vi "Start Acquisition and Logging.vi"(8 "error in (no error)":errorcluster, 11 "Acquisition and Logging Configuration":T2={"Data Rate"=1, "Samples per Read"=0, "Number of Reads to Save"=0, "Data File Name"="", "TDMS Properties"=[], "Number of Channels"=4, "Channel Scale Array"=[0.0, 0.0, 0.0, 0.0, 1.0, 1.0, 1.0, 1.0, 1.0, 1.0, 1.0, 1.0, 1.0, 1.0, 1.0, 1.0], "Channel Names"=[], "Trigger - RMS Value"=0.0, "Trigger - Channel"=0, "Trigger - Time (Minute)"=0, "Frequency "=0, "Amplitude (0~10)"=0.0} {"Amplitude (0~10)" min=-10.0 max=10.0; "Data Rate" items=["50.000 kS/s (NI 9239)"=1, "25.000 kS/s (NI 9239)"=2, "16.667 kS/s (NI 9239)"=3, "12.500 kS/s (NI 9239)"=4, "10.000 kS/s (NI 9239)"=5, "8.333 kS/s (NI 9239)"=6, "7.143 kS/s (NI 9239)"=7, "6.250 kS/s (NI 9239)"=8, "5.556 kS/s (NI 9239)"=9, "5.000 kS/s (NI 9239)"=10, "4.545 kS/s (NI 9239)"=11, "4.167 kS/s (NI 9239)"=12, "3.846 kS/s (NI 9239)"=13, "3.571 kS/s (NI 9239)"=14, "3.333 kS/s (NI 9239)"=15, "3.125 kS/s (NI 9239)"=16, "2.941 kS/s (NI 9239)"=17, "2.778 kS/s (NI 9239)"=18, "2.632 kS/s (NI 9239)"=19, "2.500 kS/s (NI 9239)"=20, "2.381 kS/s (NI 9239)"=21, "2.273 kS/s (NI 9239)"=22, "2.174 kS/s (NI 9239)"=23, "2.083 kS/s (NI 9239)"=24, "2.000 kS/s (NI 9239)"=25, "1.923 kS/s (NI 9239)"=26, "1.852 kS/s (NI 9239)"=27, "1.786 kS/s (NI 9239)"=28, "1.724 kS/s (NI 9239)"=29, "1.667 kS/s (NI 9239)"=30, "1.613 kS/s (NI 9239)"=31]}) -> (0 "error out":errorcluster, 1 "Wait on IRQ Timeout?":bool, 2 "Total Buffer Size":i32, 3 "FPGA VI Reference Out":T5)   [LabVIEW 2016]
uses:
  controls/FPGA VI Reference.ctl
  controls/Acquisition and Logging Configuration.ctl
  <vilib>/LabVIEW Targets/FPGA/cRIO/shared/nicrio_ModuleControls/nicrio_cRIO-9239_DataRatesRing.ctl
  controls/TDMS Properties.ctl
  <vilib>/userdefined/High Color/nirio_resource_hc.ctl
  <vilib>/FPGAPlugInAG/cRIO-9068/niLvFpga_Open_cRIO-9068.vi
  <vilib>/rvi/interface/common/dynamic/niFpgaDynamicAddResources.vi
  <vilib>/FPGAPlugInAG/Dynamic/niLvFpga_Reset_Dynamic.vi
  <vilib>/Utility/error.llb/Error Cluster From Error Code.vi
  <vilib>/rvi/errors/niLvFpgaAdjustHostInterfaceError.vi
  <vilib>/rvi/interface/common/niFpgaWaitOnOcc.vi
  <vilib>/FPGAPlugInAG/Dynamic/niLvFpga_Run_Dynamic.vi
  <vilib>/RVI Host/nirviSupport.llb/nirviErrorClusterFromErrorCode.vi
  <vilib>/FPGAPlugInAG/Dynamic/niLvFpga_Close_Dynamic.vi
  <vilib>/rvi/interface/nirviOpenFPGA/nirviOpenFPGA.xnode
  FPGA Bitfiles/v1.1.10032017CSU_FPGATarget2_FPGAMain_uXAbGLR-yyg.lvbitx
  FPGA Main.vi
  <vilib>/rvi/interface/nirviMethod/nirviMethod.xnode
  <vilib>/rvi/interface/nirviReadWriteControl/nirviReadWriteControl.xnode
  <vilib>/rvi/interface/nirviCloseFPGA/nirviCloseFPGA.xnode
  <vilib>/rvi/errors/niLvFpgaMergeErrorWithErrorCode.vi
  <vilib>/rvi/interface/nirviMethod/StockFPGA_InlinedMethodWaitForSingleIRQ.vi
  <vilib>/FPGAPlugInAG/Dynamic/niLvFpga_WaitOnIrq_Dynamic.vi
  <vilib>/FPGAPlugInAG/Dynamic/niLvFpga_AcknowledgeIrq_Dynamic.vi
  <vilib>/FPGAPlugInAG/Dynamic/niLvFpga_ConfigureFifo_Dynamic.vi
  <vilib>/FPGAPlugInAG/Dynamic/niLvFpga_StartFifo_Dynamic.vi
  NiFpgaLv.dll
  <vilib>/rvi/interface/Simulation/niFpgaSimulationCallBeginRW.vi
  <vilib>/FPGAPlugInAG/Dynamic/niLvFpga_WriteFifo_Dynamic.vi
  <vilib>/FPGAPlugInAG/Dynamic/niLvFpga_ReadFifo_Dynamic.vi
panel:
  in  "Sample Frequency (Hz)":dbl=1000.0
  in  "resource name":T1="RIO0" caption="RIO Device"
  in  "stop":bool
  out "AO FIFO Empty":bool
  out "AI FIFO Full":bool
  out "AI Data":dbl[][](graph)
  # "Caso o sistema esteja Ok essa VI é chamada.\nEla contém tanto a chamada para aquisição quanto para a supervisão\nOs dados anaçógicos podem ser vistos no display em colorido.\nA VI rodada separamente funciona, mas não quando for chamada dentro do programa principal \"RT Main.vi\""
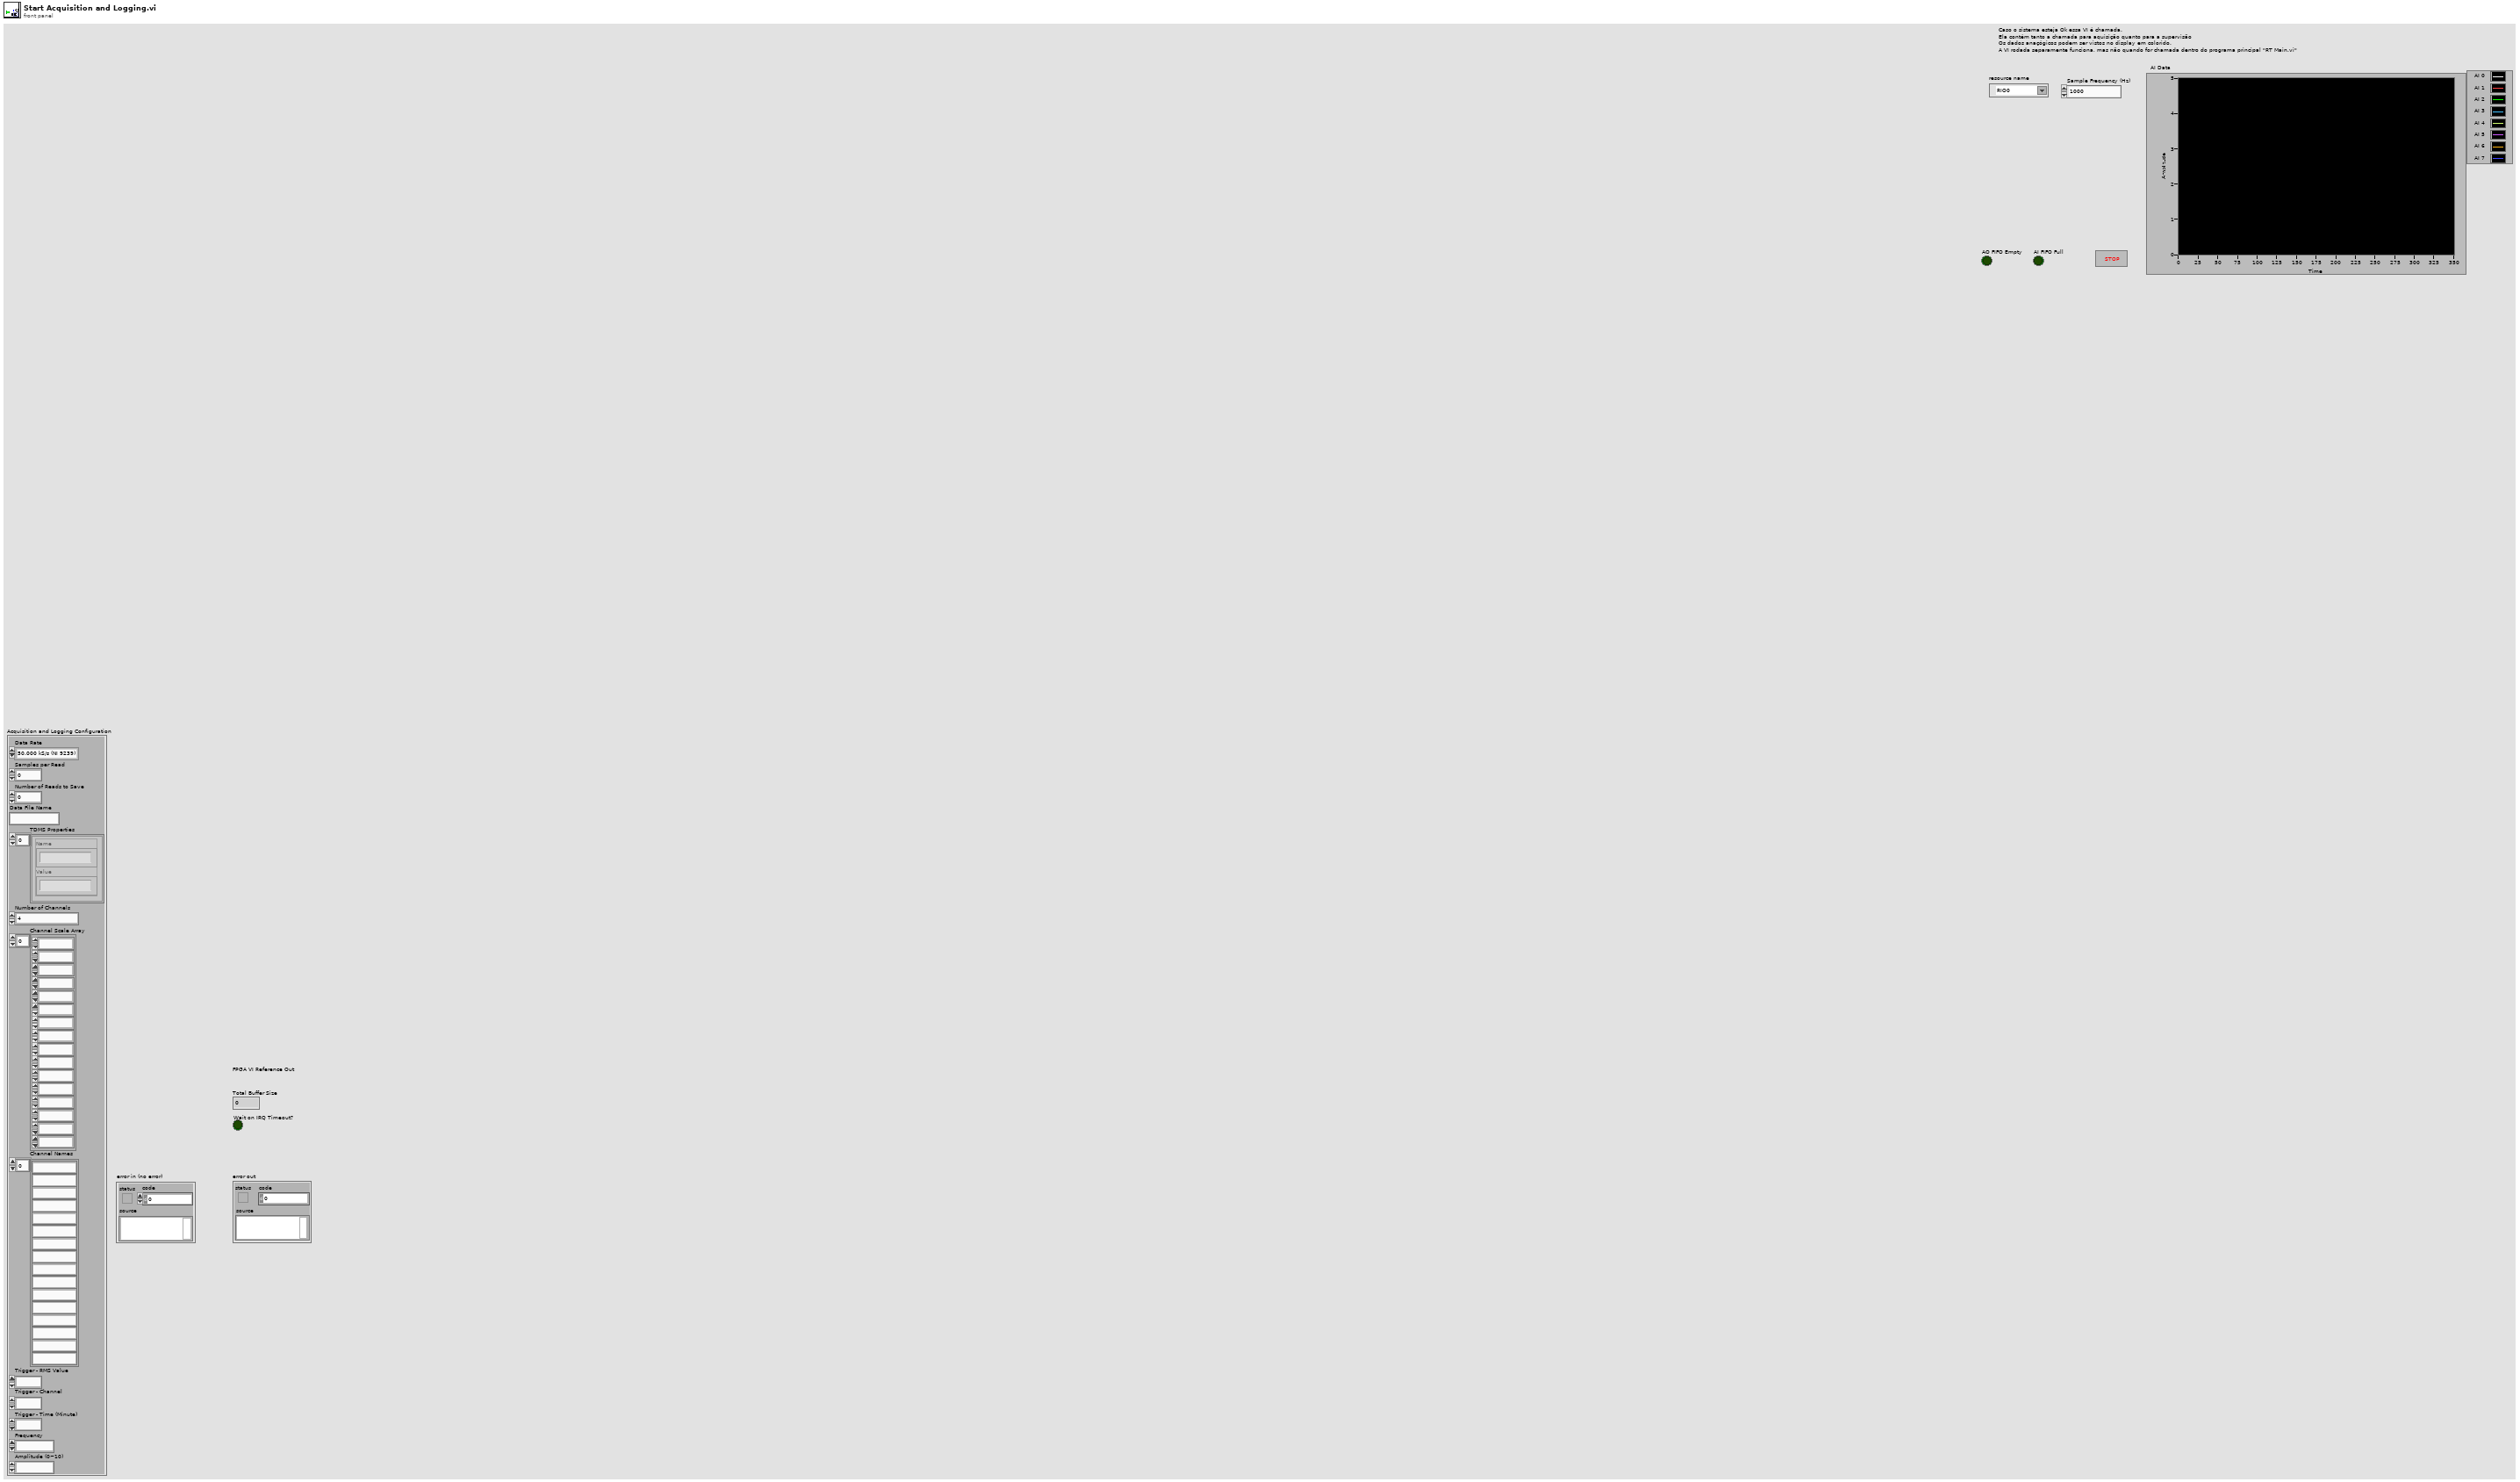
[diagram p1: front panel]
types:
  T1 = typedef "nirio_resource_hc.ctl" = tag
  T2 = typedef "Acquisition and Logging Configuration.ctl" = cluster{"Data Rate":T3, "Samples per Read":i32, "Number of Reads to Save":i32, "Data File Name":string, "TDMS Properties":T4[], "Number of Channels":i32, "Channel Scale Array":fxp<+,24,12>[], "Channel Names":string[], "Trigger - RMS Value":dbl, "Trigger - Channel":i32, "Trigger - Time (Minute)":i32, "Frequency ":i32, "Amplitude (0~10)":dbl}
  T3 = typedef "nicrio_cRIO-9239_DataRatesRing.ctl" = u8
  T4 = typedef "TDMS Properties.ctl" = cluster{"Name":string, "Value":string}
  T5 = typedef "FPGA VI Reference.ctl" = refnum<k20>
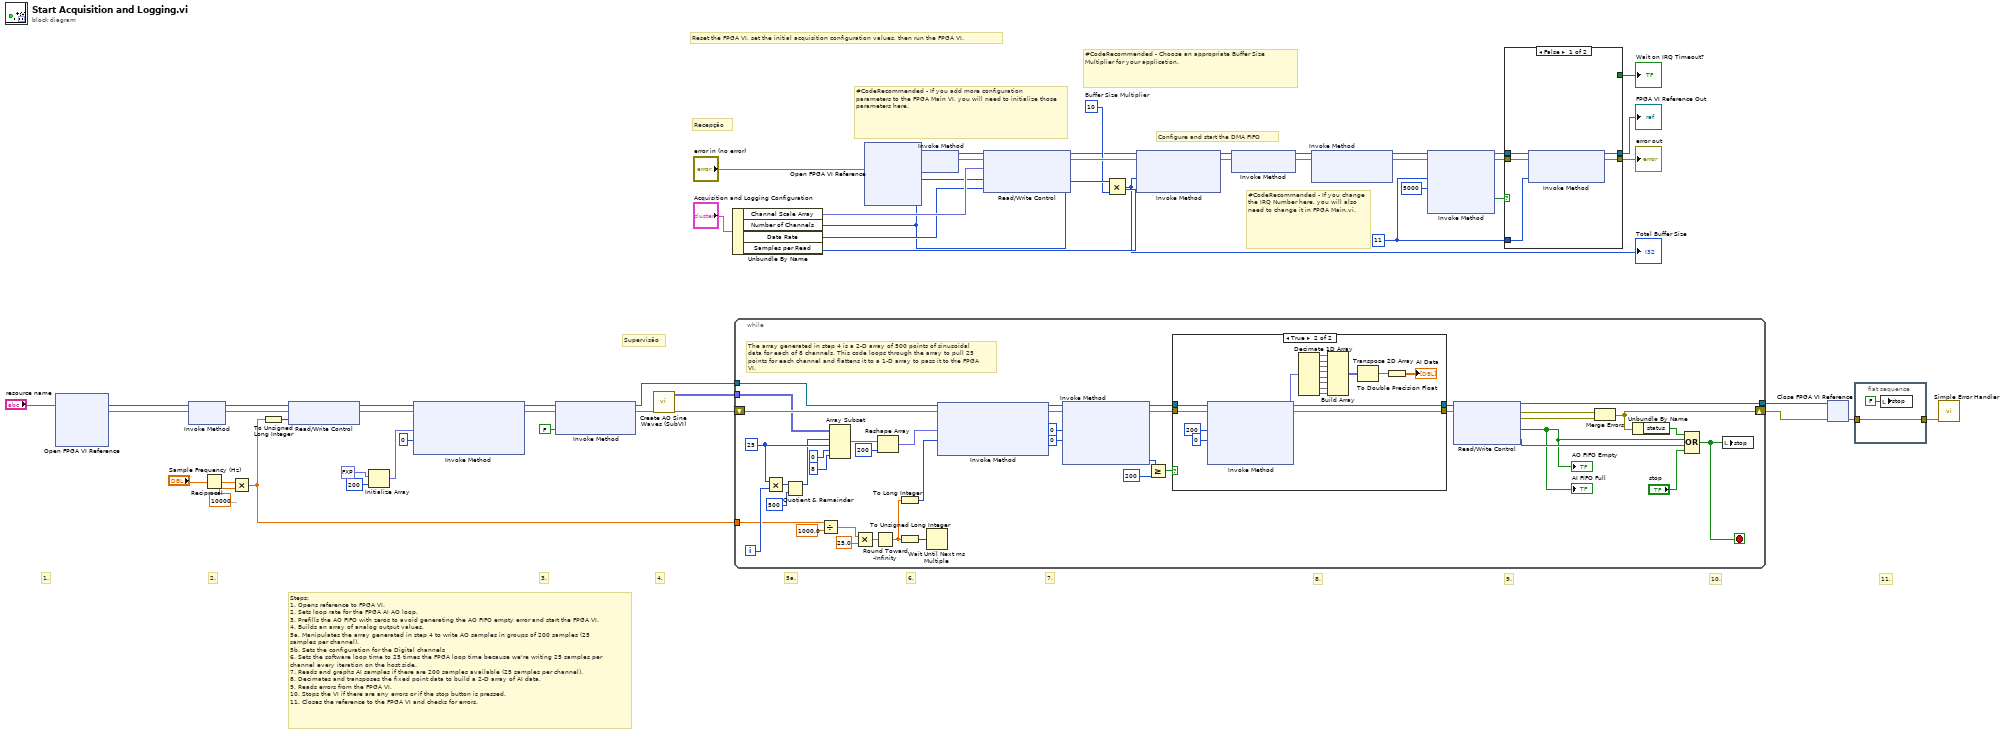
[diagram p0: block diagram]
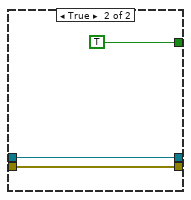
[diagram p3: hidden frame]
diagram:
  w34 = 11
  w35 = 10  # Buffer Size Multiplier
  # "11."
  # "10."
  # "9."
  # "4."
  # "2."
  # "Steps:\n1. Opens reference to FPGA VI.\n2. Sets loop rate for the FPGA AI AO loop.\n3. Prefills the AO FIFO with zeros to avoid generating the AO FIFO empty error and start the FPGA VI.\n4. Builds an array of analog output values.\n5a. Manipulates the array generated in step 4 to write AO samples in groups of 200 samples (25 samples per channel).\n5b. Sets the configuration for the Digital channels \n6. Sets the software loop time to 25 times the FPGA loop time because we're writing 25 samples per channel every iteration on the host side.\n7. Reads and graphs AI samples if there are 200 samples available (25 samples per channel).\n8. Decimates and transposes the fixed point data to build a 2-D array of AI data.\n9. Reads errors from the FPGA VI.\n10. Stops the VI if there are any errors or if the stop button is pressed.\n11. Closes the reference to the FPGA VI and checks for errors."
  # "8."
  # "7."
  # "6."
  # "5a."
  # "3."
  # "1."
  # "Supervisão"
  # "Recepção"
  # "#CodeRecommended - If you change the IRQ Number here, you will also need to change it in FPGA Main.vi."
  # "#CodeRecommended - Choose an appropriate Buffer Size Multiplier for your application."
  # "Configure and start the DMA FIFO"
  # "#CodeRecommended - If you add more configuration parameters to the FPGA Main VI, you will need to initialize those parameters here."
  # "Reset the FPGA VI, set the initial acquisition configuration values, then run the FPGA VI."
  n1 = xnode "Open FPGA VI Reference"("resource name"="resource name") -> ("FPGA VI Reference Out"=w5:refnum<k20>, "error out"=w4:errorcluster)  [unwired: 1 in]
  n2 = xnode "Invoke Method"("FPGA VI Reference In"=w5, "error in"=w4) -> ("FPGA VI Reference Out"=w7:refnum<k20>, "error out"=w6:errorcluster)
  n3 = Reciprocal(x="Sample Frequency (Hz)") -> (1/x=w23:dbl)
  n4 = Multiply(x=w23, y=1000000.0) -> (x*y=w2:dbl)
  n5 = To Unsigned Long Integer(number=w2) -> (unsigned 32bit integer=w3:u32)
  n6 = xnode "Read/Write Control"("FPGA VI Reference In"=w7, "error in"=w6, "Loop Rate(uSec)"=w3) -> ("FPGA VI Reference Out"=w12:refnum<k20>, "error out"=w13:errorcluster)
  n7 = Initialize Array(fxp<+,16,3> 0.0, 200 ("dimension size")) -> (w16:fxp<+,16,3>[])
  n8 = xnode "Invoke Method"("FPGA VI Reference In"=w12, "error in"=w13, "Data"=w16, "Timeout (ms)"=0) -> ("FPGA VI Reference Out"=w10:refnum<k20>, "error out"=w11:errorcluster)  [unwired: 1 out]
  n9 = xnode "Invoke Method"("FPGA VI Reference In"=w10, "error in"=w11, "Wait Until Done (F)"=FALSE) -> ("FPGA VI Reference Out"=w25:refnum<k20>, "error out"=w20:errorcluster)
  n10 = call "Create AO Sine Waves (SubVI).vi"("error in (no error)"=w20) -> ("error out"=w19:errorcluster, "Output Array"=w21:fxp<+,16,3>[][])  [unwired: 9 in]
  n11 = Unbundle By Name("Acquisition and Logging Configuration") -> ("Channel Scale Array"=w46:fxp<+,24,12>[], "Number of Channels"=w38:i32, "Data Rate"=w45:T3, "Samples per Read"=w37:i32)
  n12 = while {
    tunnel: w25 -> [w90]
    tunnel: [w95] -> w27
    shift-right: [w94] -> w1
    shift-left: w19 -> [w89]
    tunnel: w21 -> [w88]
    tunnel: w2 -> [w59]
    i -> [w76]
    stop <- w70 stop-if-true
    w77 = 25 ("length")
    # "The array generated in step 4 is a 2-D array of 500 points of sinusoidal data for each of 8 channels. This code loops through the array to pull 25 points for each channel and flattens it to a 1-D array to pass it to the FPGA VI."
    n13 = Multiply(x=w77, y=w76) -> (x*y=w75:i32)
    n14 = Quotient & Remainder(x=w75, y=500) -> (x-y*floor(x/y)=w73:i32)  [unwired: 1 out]
    n15 = Divide(x=w59, y=1000.0) -> (x/y=w60:dbl)
    n16 = Array Subset(array=w88, index (row)=w73, length (row)=w77, index (col)=0 ("index"), length (col)=8 ("length")) -> (w85:fxp<+,16,3>[][])
    n17 = Multiply(x=w60, y=25.0) -> (x*y=w62:dbl)
    n18 = Round Toward -Infinity(1:w62) -> (0:w56:dbl)
    n19 = Reshape Array(w85, 200 ("dimension size")) -> (w84:fxp<+,16,3>[])
    n20 = To Long Integer(number=w56) -> (32bit integer=w57:i32)
    n21 = To Unsigned Long Integer(number=w56) -> (unsigned 32bit integer=w58:u32)
    n22 = Wait Until Next ms Multiple(millisecond multiple=w58) -> ()  [unwired: 1 out]
    n23 = xnode "Invoke Method"("FPGA VI Reference In"=w90, "error in"=w89, "Data"=w84, "Timeout (ms)"=w57) -> ("FPGA VI Reference Out"=w68:refnum<k20>, "error out"=w69:errorcluster)  [unwired: 1 out]
    n24 = xnode "Invoke Method"("FPGA VI Reference In"=w68, "error in"=w69, "Number of Elements"=u32 0, "Timeout (ms)"=0) -> ("FPGA VI Reference Out"=w82:refnum<k20>, "error out"=w81:errorcluster, "Elements Remaining"=w80:u32)  [unwired: 1 out]
    n25 = Greater Or Equal?(x=w80, y=u32 200 ("Number of Elements")) -> (x >= y?=w79:bool)
    n26 = case shown="True" w79 {
      tunnel: [w98 w108] -> w93
      tunnel: [w97 w107] -> w92
      tunnel: w82 -> [w98 w102]
      tunnel: w81 -> [w97 w101]
      frame False {
      }
      frame True {
        n27 = xnode "Invoke Method"("FPGA VI Reference In"=w102, "error in"=w101, "Number of Elements"=u32 200, "Timeout (ms)"=0) -> ("FPGA VI Reference Out"=w108:refnum<k20>, "error out"=w107:errorcluster, "Data"=w104:fxp<+/-,20,5>[])  [unwired: 1 out]
        n28 = Decimate 1D Array(w104) -> (w116:fxp<+/-,20,5>[], w115:fxp<+/-,20,5>[], w114:fxp<+/-,20,5>[], w113:fxp<+/-,20,5>[], w112:fxp<+/-,20,5>[], w111:fxp<+/-,20,5>[], w110:fxp<+/-,20,5>[], w109:fxp<+/-,20,5>[])
        n29 = Build Array(w116, w115, w114, w113, w112, w111, w110, w109) -> (w105:fxp<+/-,20,5>[][])
        n30 = Transpose 2D Array(2D array=w105) -> (transposed array=w106:fxp<+/-,20,5>[][])
        n31 = To Double Precision Float(number=w106) -> (double precision float=→"AI Data":dbl[][])
      }
    }
    n32 = xnode "Read/Write Control"("FPGA VI Reference In"=w93, "error in"=w92) -> ("FPGA VI Reference Out"=w95:refnum<k20>, "error out"=w96:errorcluster, "AI AO Error"=w91:errorcluster, "AO FIFO Empty"=w63:bool, "AI FIFO Full"=w64:bool)
    "AO FIFO Empty" <- w63
    "AI FIFO Full" <- w63
    n33 = Merge Errors(w96, w91) -> (w94:errorcluster)
    n34 = Unbundle By Name(w94) -> ("status"=w72:bool)
    n35 = Compound Arithmetic op=OR(w72, w63, w64, "stop") -> (w70:bool)
    n36 = local write "stop"(w70) -> ()
  }
  n37 = xnode "Open FPGA VI Reference"("error in"="error in (no error)") -> ("FPGA VI Reference Out"=w33:refnum<k20>, "error out"=w32:errorcluster)  [unwired: 1 in]
  n38 = xnode "Invoke Method"("FPGA VI Reference In"=w33, "error in"=w32) -> ("FPGA VI Reference Out"=w28:refnum<k20>, "error out"=w29:errorcluster)
  n39 = xnode "Read/Write Control"("FPGA VI Reference In"=w28, "error in"=w29, "Channel Scale Array"=w46, "Number of Channels"=w38, "Data Rate"=w45) -> ("FPGA VI Reference Out"=w30:refnum<k20>, "error out"=w39:errorcluster)
  n40 = Compound Arithmetic op=MULTIPLY(w38, w37, w35) -> (w36:i32)
  "Total Buffer Size" <- w36
  n41 = xnode "Invoke Method"("FPGA VI Reference In"=w30, "error in"=w39, "Requested Depth"=w36) -> ("FPGA VI Reference Out"=w42:refnum<k20>, "error out"=w43:errorcluster)  [unwired: 1 out]
  n42 = xnode "Invoke Method"("FPGA VI Reference In"=w42, "error in"=w43) -> ("FPGA VI Reference Out"=w40:refnum<k20>, "error out"=w41:errorcluster)
  n43 = xnode "Invoke Method"("FPGA VI Reference In"=w40, "error in"=w41) -> ("FPGA VI Reference Out"=w53:refnum<k20>, "error out"=w54:errorcluster)  [unwired: 1 in]
  n44 = xnode "Invoke Method"("FPGA VI Reference In"=w53, "error in"=w54, "IRQ Number(s)"=w34, "Timeout (ms)"=5000) -> ("FPGA VI Reference Out"=w47:refnum<k20>, "error out"=w48:errorcluster, "Timed Out"=w50:bool)  [unwired: 1 out]
  n45 = case shown="False" w50 {
    tunnel: w47 -> [w121 w122]
    tunnel: w48 -> [w120 w124]
    tunnel: [w119 w124] -> w51
    tunnel: w34 -> [w118 _]
    tunnel: [_ TRUE] -> w52
    tunnel: [w117 w122] -> w55
    frame False {
      n46 = xnode "Invoke Method"("FPGA VI Reference In"=w121, "error in"=w120, "IRQ Number(s)"=w118) -> ("FPGA VI Reference Out"=w117:refnum<k20>, "error out"=w119:errorcluster)
    }
    frame True {
    }
  }
  "FPGA VI Reference Out" <- w55
  "Wait on IRQ Timeout?" <- w52
  "error out" <- w51
  n47 = xnode "Close FPGA VI Reference"("FPGA VI Reference In"=w27, "error in"=w1) -> ("error out"=w8:errorcluster)
  n48 = flat-sequence {
    tunnel: [w125] -> w9
    tunnel: w8 -> [w125]
    frame #0 {
      n49 = local write "stop"(FALSE ("stop")) -> ()
    }
  }
  n50 = call <vilib>:"Simple Error Handler.vi"("error in (no error)"=w9) -> ()  [unwired: 4 in, 5 out]
